vi "PicoScope4000aClose.vi"(7 "error in (no error)":errorcluster, 10 "handle in":i16) -> (0 "error out":errorcluster, 3 "handle out":i16)   [LabVIEW 2009]
doc: "This closes the oscilloscope and should be called before exiting an application."
uses:
  Program Files/Pico Technology/SDK/lib/ps4000a.dll
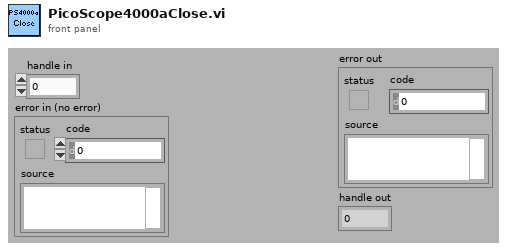
[diagram p1: front panel]
types:
  T1 = cluster{"status":bool, "code":u32, "source":string}
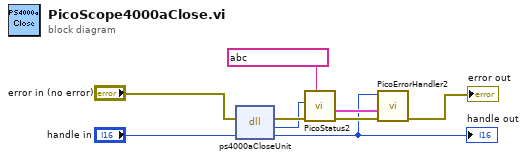
[diagram p0: block diagram]
diagram:
  n1 = dll-call lib="/Program Files/Pico Technology/SDK/lib/ps4000a.dll" fn="ps4000aCloseUnit" ("ps3000.dll:_ps3000_open_unit@0")(error in="error in (no error)", "handle"="handle in") -> (error out=w6:errorcluster, "PICO_STATUS"=w2:u32, "handle"=w1:i16)  [unwired: 2 in, 1 out]
  "handle out" <- w1
  n2 = call "PicoStatus2.vi"("PICO source"=string ?, "Error in"=w6, "PICO STATUS"=w2) -> ("error out"=w4:errorcluster, "PICO_STATUS out"=w3:T1)  [unwired: 5 in]
  n3 = call "PicoErrorHandler2.vi"("error in (no error)"=w4, "PICO_STATUS in"=w3, "handle In"=w1) -> ("error out"=→"error out":errorcluster)  [unwired: 8 in]
